vi "Test Assert Equal Value.vi"(8 "error in (no error)":errorcluster) -> (0 "error out":errorcluster)   [LabVIEW 2020]
uses:
  classes/Assert/Assert.lvclass
  classes/Test/Test.lvclass
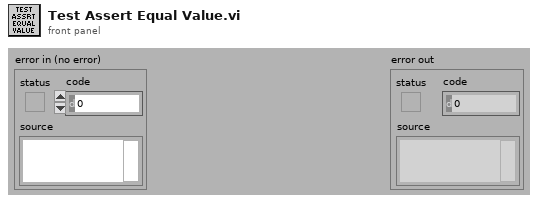
[diagram p1: front panel]
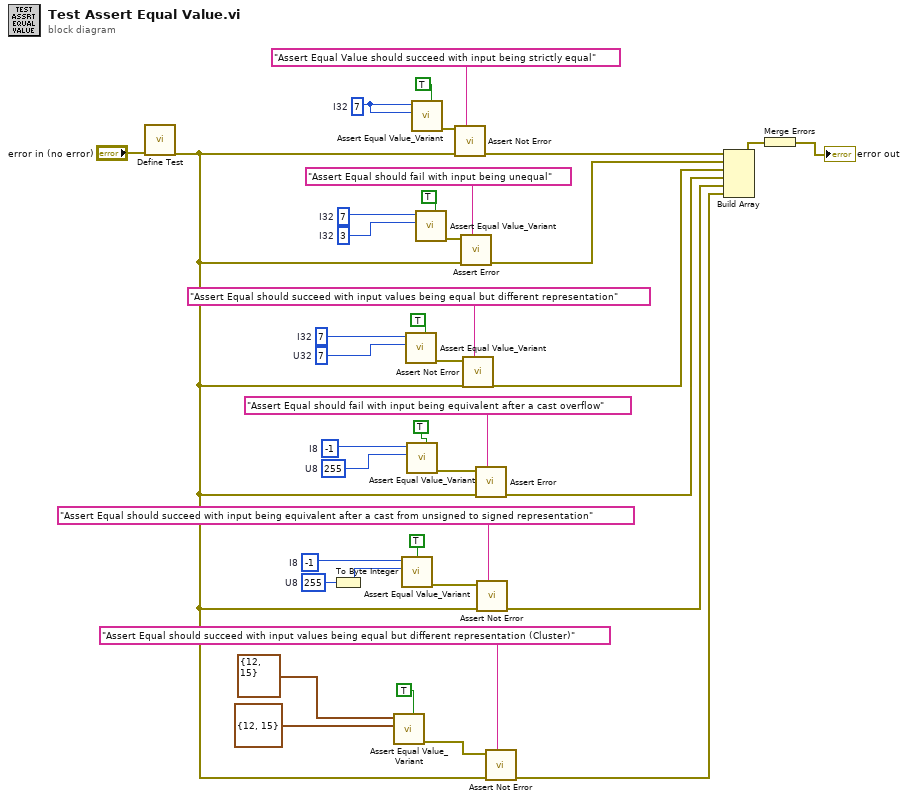
[diagram p0: block diagram]
diagram:
  w22 = 3  # I32
  w23 = 7  # I32
  w28 = 7  # I32
  w32 = u8 255  # U8
  w12 = i8 -1  # I8
  w14 = u8 255  # U8
  w15 = i8 -1  # I8
  w8 = u32 7  # U32
  w9 = 7  # I32
  n1 = call "Define Test.vi"("error in (no error)"="error in (no error)") -> ("error out"=w6:errorcluster)  [unwired: 9 in, 1 out]
  n2 = To Byte Integer(number=w32) -> (8bit integer=w11:i8)
  n3 = call "Assert Equal Value_Variant.vi"("Assert Only? (F)"=TRUE, "Y"=cluster{"Width":u32, "U32":u32} {"Width"=12, "U32"=15} ("Bounds"), "X"=cluster{"Width":u32, "I32":i32} {"Width"=12, "I32"=15} ("Bounds")) -> ("error out"=w3:errorcluster)  [unwired: 7 in, 1 out]
  n4 = call "Assert Equal Value_Variant.vi"("Assert Only? (F)"=TRUE, "Y"=w11, "X"=w12) -> ("error out"=w10:errorcluster)  [unwired: 7 in, 1 out]
  n5 = call "Assert Equal Value_Variant.vi"("Assert Only? (F)"=TRUE, "Y"=w8, "X"=w9) -> ("error out"=w20:errorcluster)  [unwired: 7 in, 1 out]
  n6 = call "Assert Equal Value_Variant.vi"("Assert Only? (F)"=TRUE, "Y"=w14, "X"=w15) -> ("error out"=w17:errorcluster)  [unwired: 7 in, 1 out]
  n7 = call "Assert Equal Value_Variant.vi"("Assert Only? (F)"=TRUE, "Y"=w28, "X"=w28) -> ("error out"=w27:errorcluster)  [unwired: 7 in, 1 out]
  n8 = call "Assert Equal Value_Variant.vi"("Assert Only? (F)"=TRUE, "Y"=w22, "X"=w23) -> ("error out"=w26:errorcluster)  [unwired: 7 in, 1 out]
  n9 = call "Assert Not Error.vi"("Label"="Assert Equal Value should succeed with input being strictly equal", "error in (no error)"=w6, "Not Error?"=w27) -> ("error out"=w36:errorcluster)  [unwired: 7 in, 1 out]
  n10 = call "Assert Error.vi"("Label"="Assert Equal should fail with input being unequal", "error in (no error)"=w6, "Error?"=w26) -> ("error out"=w35:errorcluster)  [unwired: 7 in, 1 out]
  n11 = call "Assert Not Error.vi"("Label"="Assert Equal should succeed with input values being equal but different representation", "error in (no error)"=w6, "Not Error?"=w20) -> ("error out"=w19:errorcluster)  [unwired: 7 in, 1 out]
  n12 = call "Assert Error.vi"("Label"="Assert Equal should fail with input being equivalent after a cast overflow", "error in (no error)"=w6, "Error?"=w17) -> ("error out"=w30:errorcluster)  [unwired: 7 in, 1 out]
  n13 = call "Assert Not Error.vi"("Label"="Assert Equal should succeed with input being equivalent after a cast from unsigned to signed representation", "error in (no error)"=w6, "Not Error?"=w10) -> ("error out"=w29:errorcluster)  [unwired: 7 in, 1 out]
  n14 = call "Assert Not Error.vi"("Label"="Assert Equal should succeed with input values being equal but different representation (Cluster)", "error in (no error)"=w6, "Not Error?"=w3) -> ("error out"=w1:errorcluster)  [unwired: 7 in, 1 out]
  n15 = Build Array(w36, w35, w19, w30, w29, w1) -> (w34:errorcluster[])
  n16 = Merge Errors(w34) -> (→"error out":errorcluster)
